vi "Story Catalogue.vi"() -> (2 "arcs":T1(array[cluster]), 3 "steps":T2[](array[typedef]))   [LabVIEW 2020, in "Full Featured MCP Server.lvlib"]
doc: "The stories of the market, as data. A story is a chain of steps; each step is an event (see Event Catalogue) published delay min to delay max seconds after the step before. After a step the story goes on with the step next if good or next if bad (-1 ends it); odds is the chance of the good branch for an average company, strong companies get a better chance and weak ones a worse one. arcs lists where each story starts and which stocks can play the lead (empty = any stock)."
uses:
  Full Featured MCP Server.lvlib
  Story Step.ctl
  Event Template.ctl
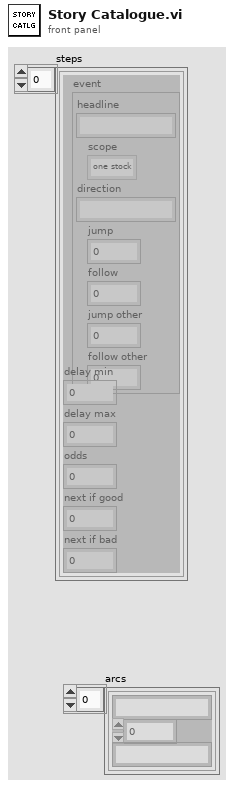
[diagram p1: front panel]
types:
  T1 = cluster{"title":string, "first step":i32, "leads":i32[]}[]
  T2 = typedef "Full Featured MCP Server.lvlib/Story Step.ctl" = cluster{"event":T3, "delay min":i32, "delay max":i32, "odds":dbl, "next if good":i32, "next if bad":i32}
  T3 = typedef "Full Featured MCP Server.lvlib/Event Template.ctl" = cluster{"headline":string, "scope":enum16{"one stock", "two stocks", "sector", "market"}, "direction":string, "jump":dbl, "follow":dbl, "jump other":dbl, "follow other":dbl}
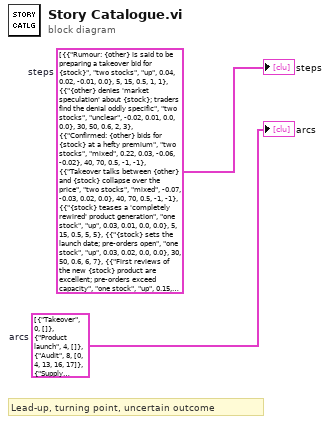
[diagram p0: block diagram]
diagram:
  w2 = T1 [{"title"="Takeover", "first step"=0, "leads"=[]}, {"title"="Product launch", "first step"=4, "leads"=[]}, {"title"="Audit", "first step"=8, "leads"=[0, 4, 13, 16, 17]}, {"title"="Supply shortage", "first step"=12, "leads"=[1, 5, 9, 10]}, {"title"="Tender", "first step"=16, "leads"=[]}, {"title"="Change at the top", "first step"=20, "leads"=[]}, {"title"="Patent suit", "first step"=23, "leads"=[]}, {"title"="Standards vote", "first step"=27, "leads"=[]}, {"title"="Interest rate decision", "first step"=31, "leads"=[]}, {"title"="Short-seller attack", "first step"=35, "leads"=[]}]  # arcs
  w1 = T2[] [{"event"={"headline"="Rumour: {other} is said to be preparing a takeover bid for {stock}", "scope"=enum."two stocks", "direction"="up", "jump"=0.04, "follow"=0.02, "jump other"=-0.01, "follow other"=0.0}, "delay min"=5, "delay max"=15, "odds"=0.5, "next if good"=1, "next if bad"=1}, {"event"={"headline"="{other} denies 'market speculation' about {stock}; traders find the denial oddly specific", "scope"=enum."two stocks", "direction"="unclear", "jump"=-0.02, "follow"=0.01, "jump other"=0.0, "follow other"=0.0}, "delay min"=30, "delay max"=50, "odds"=0.6, "next if good"=2, "next if bad"=3}, {"event"={"headline"="Confirmed: {other} bids for {stock} at a hefty premium", "scope"=enum."two stocks", "direction"="mixed", "jump"=0.22, "follow"=0.03, "jump other"=-0.06, "follow other"=-0.02}, "delay min"=40, "delay max"=70, "odds"=0.5, "next if good"=-1, "next if bad"=-1}, {"event"={"headline"="Takeover talks between {other} and {stock} collapse over the price", "scope"=enum."two stocks", "direction"="mixed", "jump"=-0.07, "follow"=-0.03, "jump other"=0.02, "follow other"=0.0}, "delay min"=40, "delay max"=70, "odds"=0.5, "next if good"=-1, "next if bad"=-1}, {"event"={"headline"="{stock} teases a 'completely rewired' product generation", "scope"=enum."one stock", "direction"="up", "jump"=0.03, "follow"=0.01, "jump other"=0.0, "follow other"=0.0}, "delay min"=5, "delay max"=15, "odds"=0.5, "next if good"=5, "next if bad"=5}, {"event"={"headline"="{stock} sets the launch date; pre-orders open", "scope"=enum."one stock", "direction"="up", "jump"=0.03, "follow"=0.02, "jump other"=0.0, "follow other"=0.0}, "delay min"=30, "delay max"=50, "odds"=0.6, "next if good"=6, "next if bad"=7}, {"event"={"headline"="First reviews of the new {stock} product are excellent; pre-orders exceed capacity", "scope"=enum."one stock", "direction"="up", "jump"=0.15, "follow"=0.06, "jump other"=0.0, "follow other"=0.0}, "delay min"=45, "delay max"=75, "odds"=0.5, "next if good"=-1, "next if bad"=-1}, {"event"={"headline"="{stock} recalls its new product days after the launch: 'unexpected behaviour on first call'", "scope"=enum."one stock", "direction"="down", "jump"=-0.18, "follow"=-0.05, "jump other"=0.0, "follow other"=0.0}, "delay min"=45, "delay max"=75, "odds"=0.5, "next if good"=-1, "next if bad"=-1}, {"event"={"headline"="Whistle-blower report questions the accounts of {stock}", "scope"=enum."one stock", "direction"="down", "jump"=-0.05, "follow"=-0.02, "jump other"=0.0, "follow other"=0.0}, "delay min"=5, "delay max"=15, "odds"=0.5, "next if good"=9, "next if bad"=9}, {"event"={"headline"="Auditor opens a formal inquiry at {stock}; findings expected shortly", "scope"=enum."one stock", "direction"="down", "jump"=-0.04, "follow"=-0.02, "jump other"=0.0, "follow other"=0.0}, "delay min"=30, "delay max"=55, "odds"=0.45, "next if good"=10, "next if bad"=11}, {"event"={"headline"="{stock} cleared: the auditor finds sloppy wiring but no fraud", "scope"=enum."one stock", "direction"="up", "jump"=0.14, "follow"=0.03, "jump other"=0.0, "follow other"=0.0}, "delay min"=45, "delay max"=80, "odds"=0.5, "next if good"=-1, "next if bad"=-1}, {"event"={"headline"="{stock} must restate three years of earnings; the finance chief resigns", "scope"=enum."one stock", "direction"="down", "jump"=-0.28, "follow"=-0.06, "jump other"=0.0, "follow other"=0.0}, "delay min"=45, "delay max"=80, "odds"=0.5, "next if good"=-1, "next if bad"=-1}, {"event"={"headline"="{sector}: suppliers warn that connectors are getting scarce", "scope"=enum."sector", "direction"="down", "jump"=-0.012, "follow"=-0.012, "jump other"=0.0, "follow other"=0.0}, "delay min"=5, "delay max"=15, "odds"=0.5, "next if good"=13, "next if bad"=13}, {"event"={"headline"="{sector}: shortage confirmed, delivery times double", "scope"=enum."sector", "direction"="down", "jump"=-0.03, "follow"=-0.024, "jump other"=0.0, "follow other"=0.0}, "delay min"=30, "delay max"=50, "odds"=0.65, "next if good"=14, "next if bad"=15}, {"event"={"headline"="{sector}: a new supplier comes on line, the shortage eases faster than feared", "scope"=enum."sector", "direction"="up", "jump"=0.048, "follow"=0.024, "jump other"=0.0, "follow other"=0.0}, "delay min"=50, "delay max"=90, "odds"=0.5, "next if good"=-1, "next if bad"=-1}, {"event"={"headline"="{sector}: the shortage drags on, production lines stand still", "scope"=enum."sector", "direction"="down", "jump"=-0.042, "follow"=-0.024, "jump other"=0.0, "follow other"=0.0}, "delay min"=50, "delay max"=90, "odds"=0.5, "next if good"=-1, "next if bad"=-1}, {"event"={"headline"="Large test-system tender: {stock} and {other} are the last two bidders", "scope"=enum."two stocks", "direction"="up", "jump"=0.02, "follow"=0.01, "jump other"=0.02, "follow other"=0.01}, "delay min"=5, "delay max"=15, "odds"=0.5, "next if good"=17, "next if bad"=17}, {"event"={"headline"="Tender decision between {stock} and {other} is imminent; insiders call it a coin toss with a slight lean", "scope"=enum."two stocks", "direction"="unclear", "jump"=0.0, "follow"=0.01, "jump other"=0.0, "follow other"=0.01}, "delay min"=35, "delay max"=55, "odds"=0.5, "next if good"=18, "next if bad"=19}, {"event"={"headline"="{stock} wins the tender; {other} goes home empty-handed", "scope"=enum."two stocks", "direction"="mixed", "jump"=0.14, "follow"=0.04, "jump other"=-0.09, "follow other"=-0.03}, "delay min"=20, "delay max"=40, "odds"=0.5, "next if good"=-1, "next if bad"=-1}, {"event"={"headline"="{other} wins the tender; {stock} goes home empty-handed", "scope"=enum."two stocks", "direction"="mixed", "jump"=-0.09, "follow"=-0.03, "jump other"=0.14, "follow other"=0.04}, "delay min"=20, "delay max"=40, "odds"=0.5, "next if good"=-1, "next if bad"=-1}, {"event"={"headline"="{stock}: chief executive steps down unexpectedly; a successor is to be named shortly", "scope"=enum."one stock", "direction"="down", "jump"=-0.06, "follow"=-0.01, "jump other"=0.0, "follow other"=0.0}, "delay min"=5, "delay max"=15, "odds"=0.5, "next if good"=21, "next if bad"=22}, {"event"={"headline"="{stock} names a respected industry veteran as chief executive; first act: a refactoring budget", "scope"=enum."one stock", "direction"="up", "jump"=0.12, "follow"=0.04, "jump other"=0.0, "follow other"=0.0}, "delay min"=40, "delay max"=70, "odds"=0.5, "next if good"=-1, "next if bad"=-1}, {"event"={"headline"="{stock} names the founder's nephew as chief executive; he 'has seen LabVIEW once'", "scope"=enum."one stock", "direction"="down", "jump"=-0.1, "follow"=-0.04, "jump other"=0.0, "follow other"=0.0}, "delay min"=40, "delay max"=70, "odds"=0.5, "next if good"=-1, "next if bad"=-1}, {"event"={"headline"="{stock} sues {other} over a patent on 'wiring things from left to right'", "scope"=enum."two stocks", "direction"="unclear", "jump"=0.02, "follow"=0.0, "jump other"=-0.03, "follow other"=0.0}, "delay min"=5, "delay max"=15, "odds"=0.5, "next if good"=24, "next if bad"=24}, {"event"={"headline"="Court hearing {stock} v. {other}: the judge asks pointed questions, of both sides", "scope"=enum."two stocks", "direction"="unclear", "jump"=0.0, "follow"=0.0, "jump other"=0.0, "follow other"=0.0}, "delay min"=35, "delay max"=60, "odds"=0.5, "next if good"=25, "next if bad"=26}, {"event"={"headline"="Court rules for {stock}: {other} must pay damages and licence fees", "scope"=enum."two stocks", "direction"="mixed", "jump"=0.12, "follow"=0.03, "jump other"=-0.13, "follow other"=-0.03}, "delay min"=40, "delay max"=70, "odds"=0.5, "next if good"=-1, "next if bad"=-1}, {"event"={"headline"="Court throws out the suit: {stock} bears all costs, {other} is relieved", "scope"=enum."two stocks", "direction"="mixed", "jump"=-0.09, "follow"=-0.03, "jump other"=0.08, "follow other"=0.02}, "delay min"=40, "delay max"=70, "odds"=0.5, "next if good"=-1, "next if bad"=-1}, {"event"={"headline"="{sector}: standards committee considers making the sector's interface mandatory", "scope"=enum."sector", "direction"="up", "jump"=0.012, "follow"=0.006, "jump other"=0.0, "follow other"=0.0}, "delay min"=5, "delay max"=15, "odds"=0.5, "next if good"=28, "next if bad"=28}, {"event"={"headline"="{sector}: committee vote scheduled; lobbyists sound confident", "scope"=enum."sector", "direction"="up", "jump"=0.012, "follow"=0.012, "jump other"=0.0, "follow other"=0.0}, "delay min"=35, "delay max"=55, "odds"=0.55, "next if good"=29, "next if bad"=30}, {"event"={"headline"="{sector}: standard adopted, every test bench will need the sector's products", "scope"=enum."sector", "direction"="up", "jump"=0.054, "follow"=0.03, "jump other"=0.0, "follow other"=0.0}, "delay min"=45, "delay max"=75, "odds"=0.5, "next if good"=-1, "next if bad"=-1}, {"event"={"headline"="{sector}: committee picks a rival interface; the sector has to adapt", "scope"=enum."sector", "direction"="down", "jump"=-0.048, "follow"=-0.024, "jump other"=0.0, "follow other"=0.0}, "delay min"=45, "delay max"=75, "odds"=0.5, "next if good"=-1, "next if bad"=-1}, {"event"={"headline"="Market: central bank announces a rate decision for its next meeting", "scope"=enum."market", "direction"="unclear", "jump"=-0.003, "follow"=0.0, "jump other"=0.0, "follow other"=0.0}, "delay min"=5, "delay max"=15, "odds"=0.5, "next if good"=32, "next if bad"=32}, {"event"={"headline"="Market: economists are split on the rate decision; trading turns nervous", "scope"=enum."market", "direction"="unclear", "jump"=-0.005, "follow"=0.0, "jump other"=0.0, "follow other"=0.0}, "delay min"=35, "delay max"=55, "odds"=0.5, "next if good"=33, "next if bad"=34}, {"event"={"headline"="Market: rates cut by half a point; the exchange lights up like a front panel", "scope"=enum."market", "direction"="up", "jump"=0.025, "follow"=0.015, "jump other"=0.0, "follow other"=0.0}, "delay min"=40, "delay max"=60, "odds"=0.5, "next if good"=-1, "next if bad"=-1}, {"event"={"headline"="Market: rates raised; investors reach for the abort button", "scope"=enum."market", "direction"="down", "jump"=-0.025, "follow"=-0.015, "jump other"=0.0, "follow other"=0.0}, "delay min"=40, "delay max"=60, "odds"=0.5, "next if good"=-1, "next if bad"=-1}, {"event"={"headline"="Short-seller publishes a dossier on {stock}: 'a state machine without an exit state'", "scope"=enum."one stock", "direction"="down", "jump"=-0.12, "follow"=0.0, "jump other"=0.0, "follow other"=0.0}, "delay min"=5, "delay max"=15, "odds"=0.5, "next if good"=36, "next if bad"=36}, {"event"={"headline"="{stock} promises a detailed rebuttal with audited numbers", "scope"=enum."one stock", "direction"="up", "jump"=0.03, "follow"=0.0, "jump other"=0.0, "follow other"=0.0}, "delay min"=30, "delay max"=50, "odds"=0.5, "next if good"=37, "next if bad"=38}, {"event"={"headline"="{stock} rebuttal convinces: an independent audit confirms the numbers, short-sellers scramble to cover", "scope"=enum."one stock", "direction"="up", "jump"=0.17, "follow"=0.03, "jump other"=0.0, "follow other"=0.0}, "delay min"=40, "delay max"=70, "odds"=0.5, "next if good"=-1, "next if bad"=-1}, {"event"={"headline"="{stock} rebuttal falls flat: key numbers 'could not be reproduced'", "scope"=enum."one stock", "direction"="down", "jump"=-0.14, "follow"=-0.05, "jump other"=0.0, "follow other"=0.0}, "delay min"=40, "delay max"=70, "odds"=0.5, "next if good"=-1, "next if bad"=-1}]  # steps
  # "Lead-up, turning point, uncertain outcome"
  "steps" <- w1
  "arcs" <- w2
